vi "VIH Project Tree - Item Tag - Parse.vi"(11 "Tree Item Tag":string) -> (2 "Item File Path":path, 3 "Item Type":T1, 5 "Not Found":bool)   [LabVIEW 2014]
doc: "::: VI Helpeks :::\nCopyright (c) 2000-2026 Konstantin Shifershteyn. All rights reserved."
uses:
  VIH Project Tree Typedef - Tree Item Type.ctl
panel:
  # "VI Helpeks\nCopyright (c) 2012-2026 Konstantin Shifershteyn"
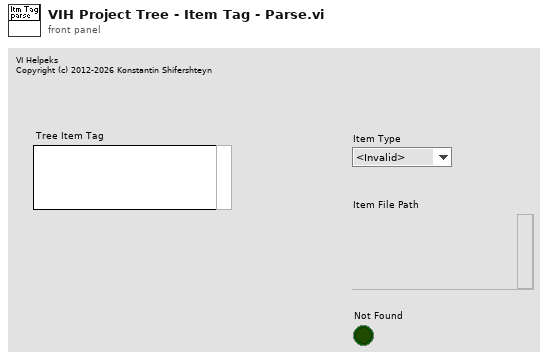
[diagram p1: front panel]
types:
  T1 = typedef "VIH Project Tree Typedef - Tree Item Type.ctl" = enum32{"<Invalid>", "Project", "Proj Files", "Proj Rules", "File Group", "Rule Group", "Any File", "LV Func", ".mnu", ".mnu (dyn)", ".vi", ".vi (dyn)", ".vit", ".vit (dyn)", ".ctl", ".ctl (dyn)", ".ctt", ".ctt (dyn)", "polyVI", "polyVI (dyn)", "expVI", "expVI (dyn)", "HTML", "PolyVI Inst"}
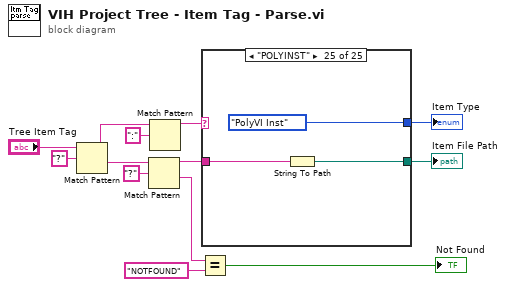
[diagram p0: block diagram]
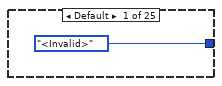
[diagram p2: hidden frame]
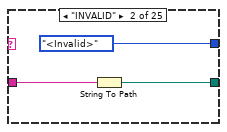
[diagram p3: hidden frame]
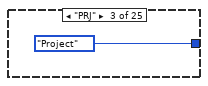
[diagram p4: hidden frame]
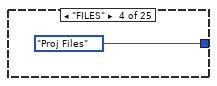
[diagram p5: hidden frame]
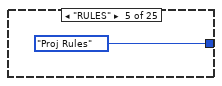
[diagram p6: hidden frame]
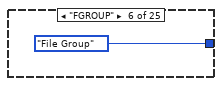
[diagram p7: hidden frame]
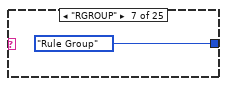
[diagram p8: hidden frame]
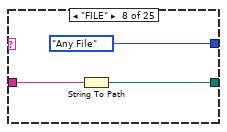
[diagram p9: hidden frame]
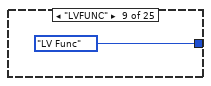
[diagram p10: hidden frame]
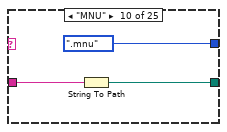
[diagram p11: hidden frame]
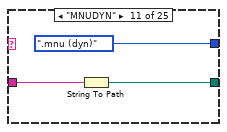
[diagram p12: hidden frame]
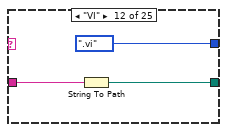
[diagram p13: hidden frame]
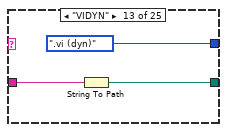
[diagram p14: hidden frame]
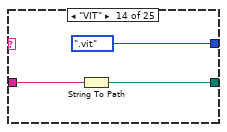
[diagram p15: hidden frame]
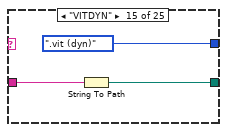
[diagram p16: hidden frame]
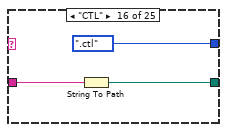
[diagram p17: hidden frame]
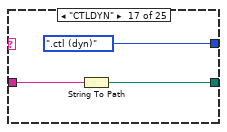
[diagram p18: hidden frame]
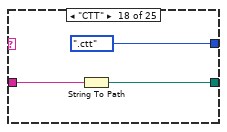
[diagram p19: hidden frame]
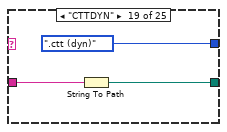
[diagram p20: hidden frame]
diagram:
  n1 = Match Pattern(string="Tree Item Tag", regular expression="?") -> (before substring=w10:string, after substring=w5:string)  [unwired: 1 in, 2 out]
  n2 = Match Pattern(string=w5, regular expression="?") -> (before substring=w4:string, after substring=w3:string)  [unwired: 1 in, 2 out]
  n3 = Match Pattern(string=w10, regular expression=":") -> (before substring=w9:string)  [unwired: 1 in, 3 out]
  n4 = Equal?(x=w3, y="NOTFOUND") -> (x = y?=→"Not Found":bool)
  n5 = case shown="\"POLYINST\"" w9 {
    tunnel: w4 -> [_ w16 _ _ _ _ _ w25 _ w29 w32 w35 w38 w41 w44 w47 w50 w53 w56 w59 w62 w65 w68 w70 w73]
    tunnel: [_ w15 _ _ _ _ _ w24 _ w28 w31 w34 w37 w40 w43 w46 w49 w52 w55 w58 w61 w64 w67 w69 w72] -> w8
    tunnel: [VIH_Project_Tree_Typedef_-_Tree_Item_Type."<Invalid>" ("Item Type") VIH_Project_Tree_Typedef_-_Tree_Item_Type."<Invalid>" ("Item Type") VIH_Project_Tree_Typedef_-_Tree_Item_Type."Project" ("Item Type") VIH_Project_Tree_Typedef_-_Tree_Item_Type."Proj Files" ("Item Type") VIH_Project_Tree_Typedef_-_Tree_Item_Type."Proj Rules" ("Item Type") VIH_Project_Tree_Typedef_-_Tree_Item_Type."File Group" ("Item Type") VIH_Project_Tree_Typedef_-_Tree_Item_Type."Rule Group" ("Item Type") VIH_Project_Tree_Typedef_-_Tree_Item_Type."Any File" ("Item Type") VIH_Project_Tree_Typedef_-_Tree_Item_Type."LV Func" ("Item Type") VIH_Project_Tree_Typedef_-_Tree_Item_Type.".mnu" ("Item Type") VIH_Project_Tree_Typedef_-_Tree_Item_Type.".mnu (dyn)" ("Item Type") VIH_Project_Tree_Typedef_-_Tree_Item_Type.".vi" ("Item Type") VIH_Project_Tree_Typedef_-_Tree_Item_Type.".vi (dyn)" ("Item Type") VIH_Project_Tree_Typedef_-_Tree_Item_Type.".vit" ("Item Type") VIH_Project_Tree_Typedef_-_Tree_Item_Type.".vit (dyn)" ("Item Type") VIH_Project_Tree_Typedef_-_Tree_Item_Type.".ctl" ("Item Type") VIH_Project_Tree_Typedef_-_Tree_Item_Type.".ctl (dyn)" ("Item Type") VIH_Project_Tree_Typedef_-_Tree_Item_Type.".ctt" ("Item Type") VIH_Project_Tree_Typedef_-_Tree_Item_Type.".ctt (dyn)" ("Item Type") VIH_Project_Tree_Typedef_-_Tree_Item_Type."polyVI" ("Item Type") VIH_Project_Tree_Typedef_-_Tree_Item_Type."polyVI (dyn)" ("Item Type") VIH_Project_Tree_Typedef_-_Tree_Item_Type."expVI" ("Item Type") VIH_Project_Tree_Typedef_-_Tree_Item_Type."expVI (dyn)" ("Item Type") VIH_Project_Tree_Typedef_-_Tree_Item_Type."HTML" ("Item Type") VIH_Project_Tree_Typedef_-_Tree_Item_Type."PolyVI Inst" ("Item Type")] -> w7
    frame Default {
    }
    frame "INVALID" {
      n6 = String To Path(string=w16) -> (path=w15:path)
    }
    frame "PRJ" {
    }
    frame "FILES" {
    }
    frame "RULES" {
    }
    frame "FGROUP" {
    }
    frame "RGROUP" {
    }
    frame "FILE" {
      n7 = String To Path(string=w25) -> (path=w24:path)
    }
    frame "LVFUNC" {
    }
    frame "MNU" {
      n8 = String To Path(string=w29) -> (path=w28:path)
    }
    frame "MNUDYN" {
      n9 = String To Path(string=w32) -> (path=w31:path)
    }
    frame "VI" {
      n10 = String To Path(string=w35) -> (path=w34:path)
    }
    frame "VIDYN" {
      n11 = String To Path(string=w38) -> (path=w37:path)
    }
    frame "VIT" {
      n12 = String To Path(string=w41) -> (path=w40:path)
    }
    frame "VITDYN" {
      n13 = String To Path(string=w44) -> (path=w43:path)
    }
    frame "CTL" {
      n14 = String To Path(string=w47) -> (path=w46:path)
    }
    frame "CTLDYN" {
      n15 = String To Path(string=w50) -> (path=w49:path)
    }
    frame "CTT" {
      n16 = String To Path(string=w53) -> (path=w52:path)
    }
    frame "CTTDYN" {
      n17 = String To Path(string=w56) -> (path=w55:path)
    }
    frame "POLYVI" {
      n18 = String To Path(string=w59) -> (path=w58:path)
    }
    frame "POLYVIDYN" {
      n19 = String To Path(string=w62) -> (path=w61:path)
    }
    frame "EXPVI" {
      n20 = String To Path(string=w65) -> (path=w64:path)
    }
    frame "EXPVIDYN" {
      n21 = String To Path(string=w68) -> (path=w67:path)
    }
    frame "HTML" {
      n22 = String To Path(string=w70) -> (path=w69:path)
    }
    frame "POLYINST" {
      n23 = String To Path(string=w73) -> (path=w72:path)
    }
  }
  "Item File Path" <- w8
  "Item Type" <- w7
